vi "Supported Protocol Versions.vi"() -> (1 "all versions":string[](array[string])=["2026-07-28", "2025-11-25", "2025-06-18", "2025-03-26", "2024-11-05"], 2 "modern versions":string[](array[string])=["2026-07-28"], 3 "supported versions":string[](array[string]))   [LabVIEW 2020, in "MCP Server.lvlib"]
doc: "The single source of the MCP protocol versions this server supports, in two eras.\n\n- supported versions: the legacy versions, negotiated by initialize.\n- modern versions: the versions served without initialize, chosen per request by params._meta.io.modelcontextprotocol/protocolVersion (2026-07-28 and later).\n- all versions: modern versions followed by supported versions, for the MCP-Protocol-Version header check, server/discover and the -32022 Unsupported protocol version error."
uses:
  MCP Server.lvlib
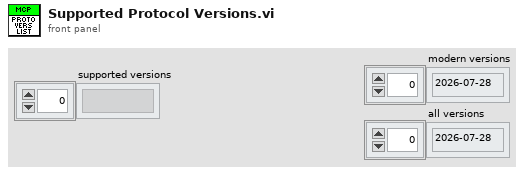
[diagram p1: front panel]
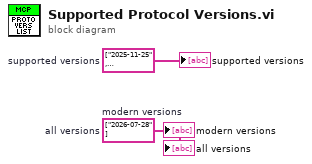
[diagram p0: block diagram]
diagram:
  w1 = string[] ["2026-07-28", "2025-11-25", "2025-06-18", "2025-03-26", "2024-11-05"]  # all versions
  w2 = string[] ["2026-07-28"]  # modern versions
  w3 = string[] ["2025-11-25", "2025-06-18", "2025-03-26", "2024-11-05"]  # supported versions
  "supported versions" <- w3
  "modern versions" <- w2
  "all versions" <- w1
